vi "Button Pressed.vi"(8 "error in (no error)":errorcluster, 9 "Data":variant, 10 "Button":T1, 11 "Guardian in":refnum<class "Guardian.lvclass">) -> (0 "error out":errorcluster, 3 "Guardian out":refnum<class "Guardian.lvclass">)   [LabVIEW 2020, in "TALOS.lvlib" / "Guardian.lvlib" / "Guardian.lvclass"]
doc: "This VI execute when a message Button Pressed is invoked from the Guardian Interface (not the GUI, the Interface...)."
uses:
  Guardian.lvclass
  C:/LabVIEW Code/TALOS/builds/Actor Framework PPL/Actor Framework.lvlibp/1abvi3w/vi.lib/ActorFramework/Actor/Actor.lvclass
  C:/LabVIEW Code/TALOS/talos/Ancestor/Ancestor/Ancestor.lvclass
  Buttons_UI.ctl
  Internal uServices/System uServices/Guardian Subpanel/Launch uService Message.ctl
  Guardian Messages/Launch uService Msg/Launch uService Msg.lvclass/Launch uService Msg.ctl
  Ancestor/Ancestor/Ancestor.lvclass/Ancestor.ctl
  Classes/uService List/uService List.lvclass/uService List.ctl
  builds/Actor Framework PPL/Actor Framework.lvlibp/1abvi3w/vi.lib/ActorFramework/Message Enqueuer/Message Enqueuer.lvclass
  Guardian.lvclass/Guardian.ctl
  Guardian Messages/Message to Other Guardian Msg/Message to Other Guardian Msg.lvclass/Message to Other Guardian Msg.ctl
  Guardian Messages/TCP-SV Message Interpreter Msg/TCP-SV Message Interpreter Msg.lvclass/TCP-SV Message Interpreter Msg.ctl
  Git Update Cluster.ctl
  Guardian Messages/Message to uService Msg/Message to uService Msg.lvclass/Message to uService Msg.ctl
  Classes/uService List/Get Queue.vi
  Ancestor/Ancestor/Read ID.vi
  Support VIs/Search Array of Strings.vi
  Guardian Messages/TCP-SV Message Interpreter Msg/Send TCP-SV Message Interpreter.vi
  FGV/Error Memory/Get Error Description.vi
  Support VIs/Get PC name.vi
  Support VIs/Get Class Name.vi
  <vilib>/Utility/error.llb/Clear Errors.vi
  FGV/Error Memory/Error Memory Core.vi
  <vilib>/AdvancedString/Delimited String to 1D String Array.vi
  FGV/Error Memory/Error Crt Lvl checker.vi
  FGV/Error Memory/Error Memory Core.vi/40c8088d-b597-4017-91af-faa98e00292e.vi
  FGV/Error Memory/Error Memory Core.vi/d4a3ab98-063c-4e44-b43d-fbdcfe6c2be2.vi
  builds/Actor Framework PPL/Actor Framework.lvlibp/1abvi3w/vi.lib/ActorFramework/Message Enqueuer/Enqueue.vi
  Support VIs/Global Memory.vi
  <vilib>/Utility/LVClass/Get LV Class Name.vi
  Support VIs/Is in Packed Library.vi
  Support VIs/TALOS Root path.vi
  Support VIs/Read CSV worksheet.vi
  Support VIs/Global Constants.vi
  <vilib>/Utility/error.llb/General Error Handler.vi
  Support VIs/Error Log.vi
  Support VIs/Circus Critical PCs List.vi
  Extract uService List from CSV.vi
  Guardian Messages/Launch uService Msg/Launch uService Msg.lvclass
  Ancestor/Ancestor/Ancestor.lvclass
  <vilib>/Comparison/Equal/Equal Functor/Equal Functor.lvclass
  Guardian Messages/Message to Other Guardian Msg/Message to Other Guardian Msg.lvclass
  Guardian Messages/TCP-SV Message Interpreter Msg/TCP-SV Message Interpreter Msg.lvclass
  Guardian Messages/Message to uService Msg/Message to uService Msg.lvclass
  Guardian Messages/I Exist Msg/I Exist Msg.lvclass
  Classes/Guardian List/Guardian List.lvclass
  Classes/uService List/uService List.lvclass
  builds/Actor Framework PPL/Actor Framework.lvlibp/1abvi3w/vi.lib/ActorFramework/Actor/Actor.lvclass
  builds/Actor Framework PPL/Actor Framework.lvlibp/1abvi3w/vi.lib/ActorFramework/Stop Msg/Stop Msg.lvclass
  TALOS.lvlib
  Internal uServices/System uServices/Guardian Subpanel/Guardian Subpanel.lvclass
  C:/LabVIEW Code/TALOS/talos/Guardian/Guardian/Guardian.lvclass
  Guardian Messages/Button Pressed Msg/Button Pressed Msg.lvclass
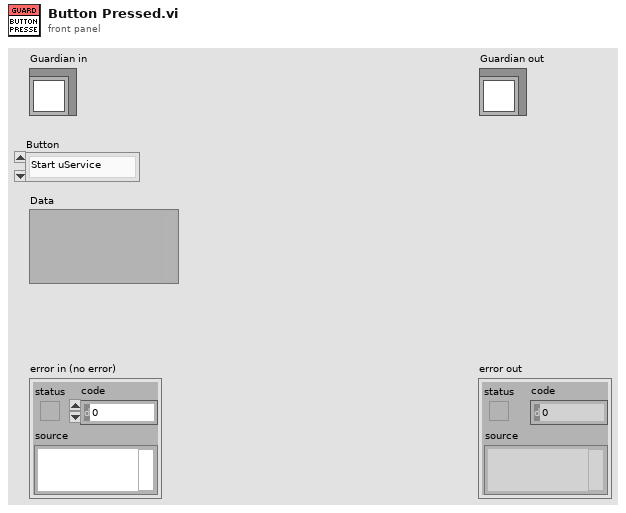
[diagram p1: front panel]
types:
  T1 = typedef "TALOS.lvlib/Guardian.lvlib/Guardian.lvclass/Buttons_UI.ctl" = enum16{"Start uService", "Kill uService", "Stop uService", "Stop", "Start online checks", "Stop online checks", "Send Pat to all GDs", "Reload INI files", "Update from GIT", "RUN", "Reset ABORT", "Check Bearer", "Send I Exist", "Change Run Config", "Add uSs from Config", "Realign uSs from Config", "Send Run Config to GD"}
  T2 = typedef "TALOS.lvlib/Guardian Subpanel.lvlib/Guardian Subpanel.lvclass/Launch uService Message.ctl" = cluster{"uService Class Name":string, "uService ID":string}
  T3 = typedef "TALOS.lvlib/Guardian.lvlib/Guardian.lvclass/Git Update Cluster.ctl" = cluster{"branch name":string, "include critical PCs":bool, "update from git":bool}
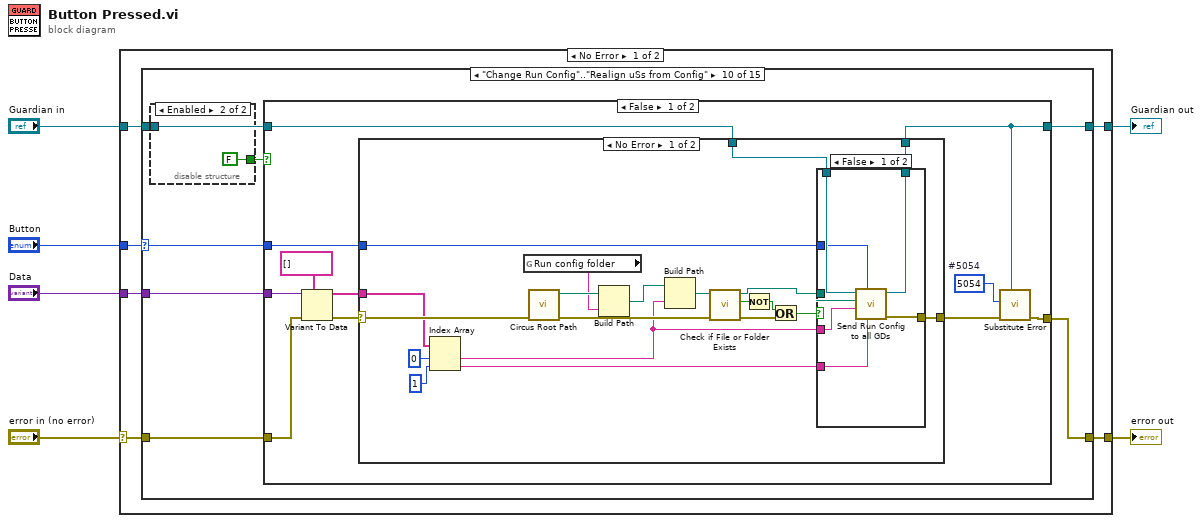
[diagram p0: block diagram]
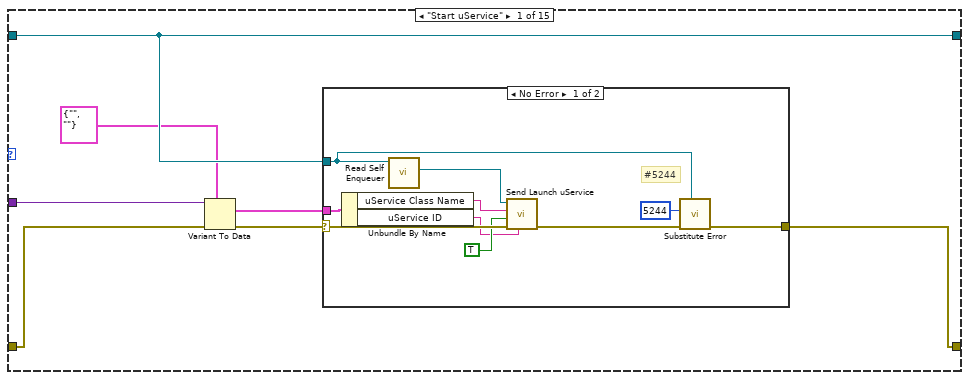
[diagram p2: hidden frame]
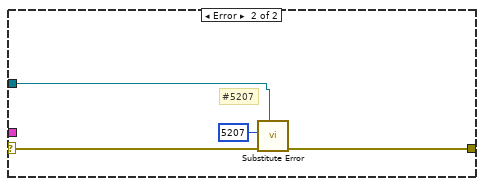
[diagram p3: hidden frame]
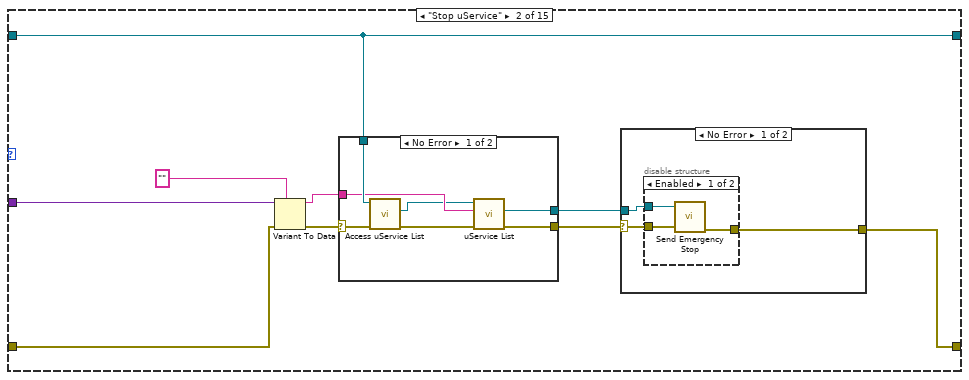
[diagram p4: hidden frame]
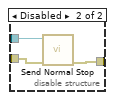
[diagram p5: hidden frame]
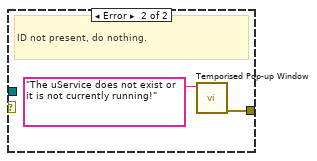
[diagram p6: hidden frame]
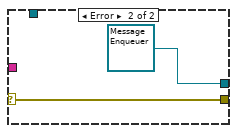
[diagram p7: hidden frame]
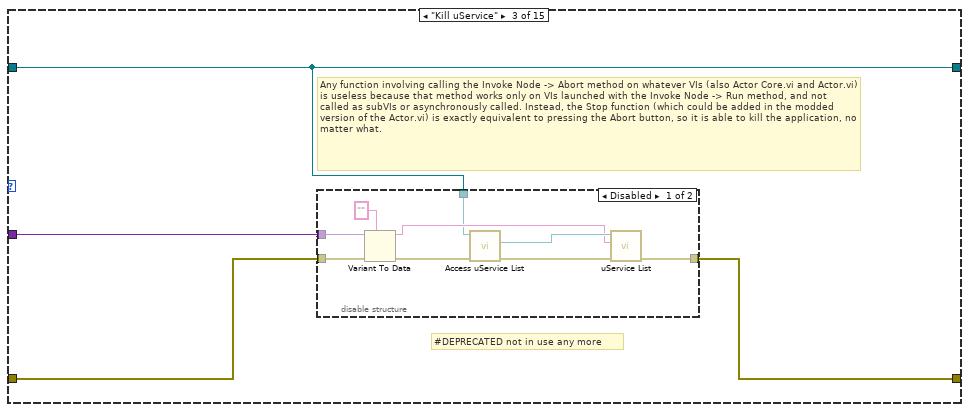
[diagram p8: hidden frame]
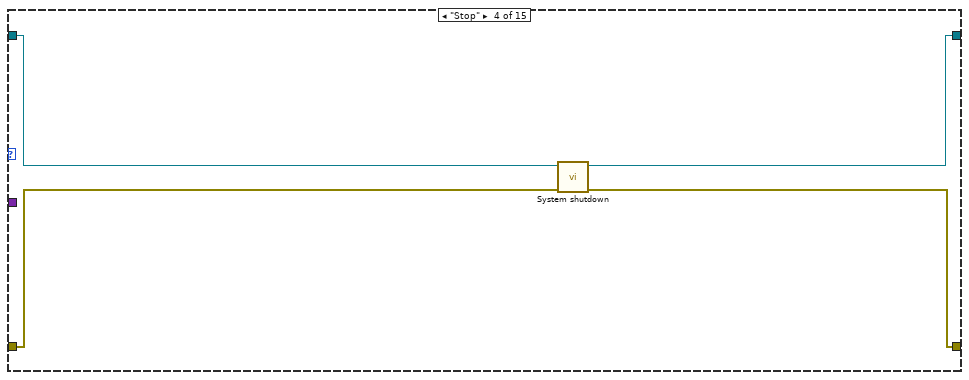
[diagram p10: hidden frame]
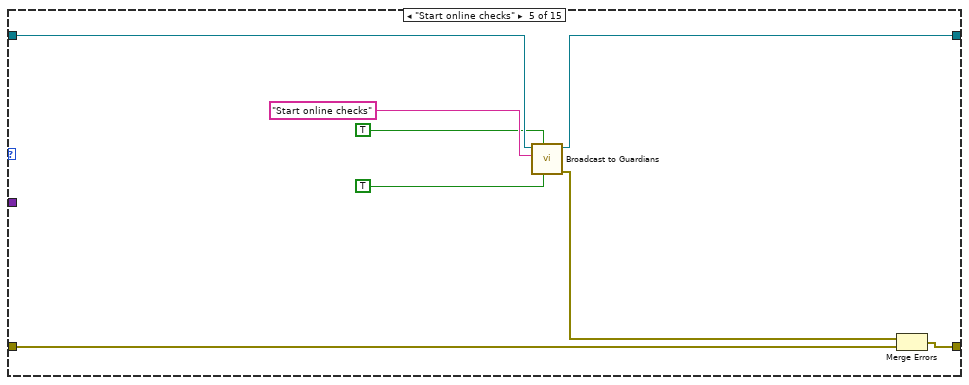
[diagram p11: hidden frame]
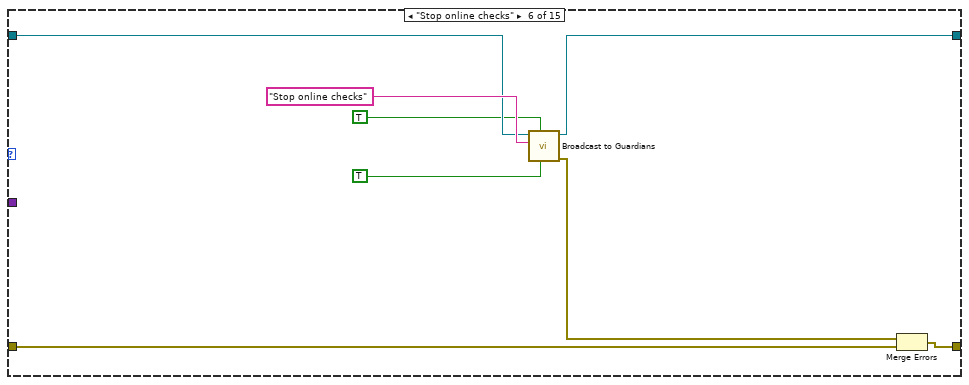
[diagram p12: hidden frame]
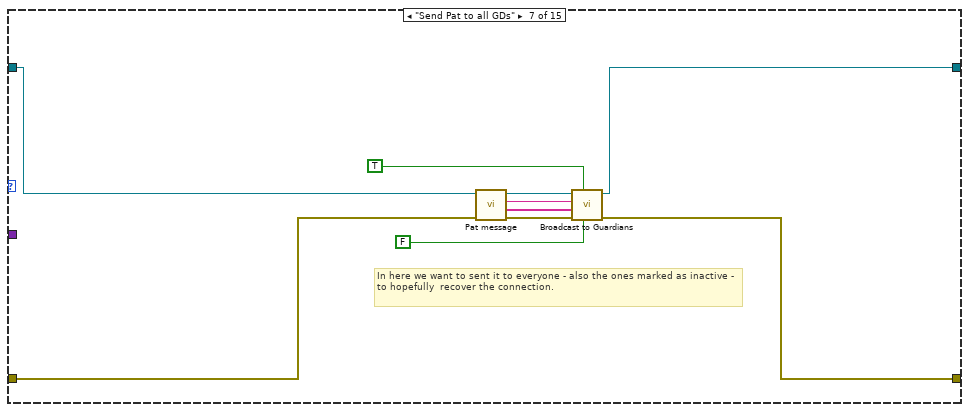
[diagram p13: hidden frame]
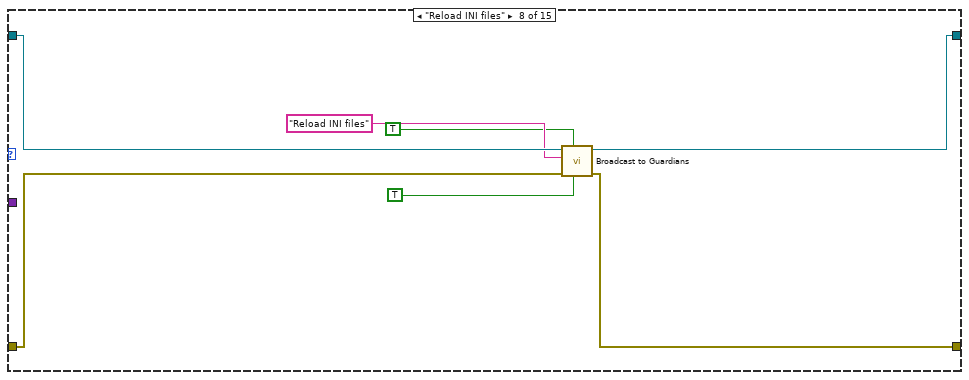
[diagram p14: hidden frame]
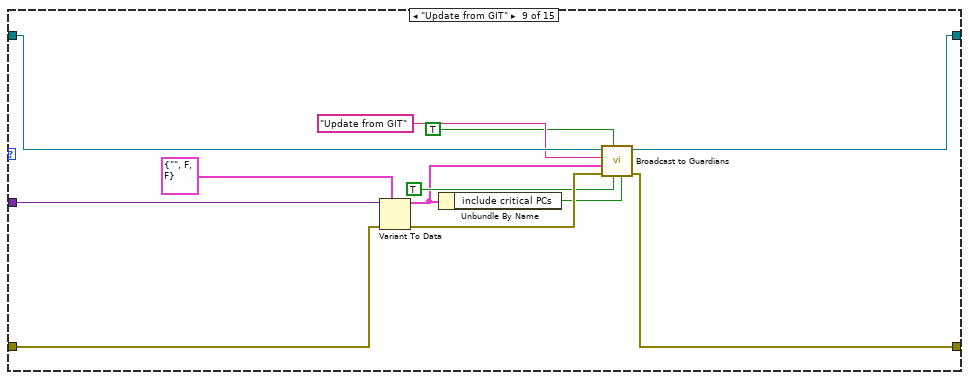
[diagram p15: hidden frame]
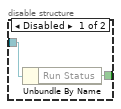
[diagram p16: hidden frame]
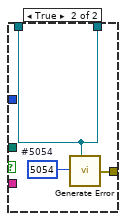
[diagram p17: hidden frame]
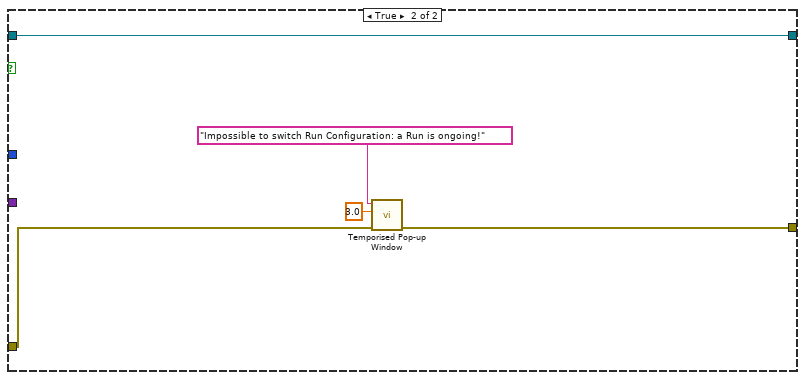
[diagram p19: hidden frame]
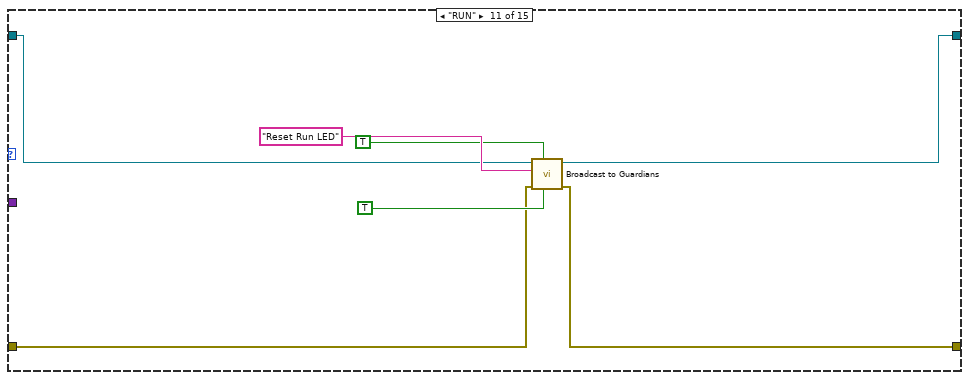
[diagram p20: hidden frame]
diagram:
  n1 = case shown="No Error" "error in (no error)" {
    selector: "error in (no error)" -> [w11 w234]
    tunnel: [w12 w234] -> w5
    tunnel: "Button" -> [w10 _]
    tunnel: [w9 w235] -> w3
    tunnel: "Guardian in" -> [w8 w235]
    tunnel: "Data" -> [w7 _]
    frame No Error {
      n2 = case shown="\"Change Run Config\"..\"Realign uSs from Config\"" w10 {
        selector: w10 -> [_ _ _ _ _ _ _ _ _ w126 _ _ _ _ _]
        tunnel: [w14 w34 w64 w80 w86 w95 w97 w108 w123 w130 w184 w196 w197 w212 w218] -> w12
        tunnel: w11 -> [w18 w41 w65 w77 w87 w96 w99 w110 w122 w132 w185 w195 _ w209 w222]
        tunnel: [w15 w38 w63 w79 w84 w91 w98 w111 w124 w129 w186 w193 w199 w213 w215] -> w9
        tunnel: w8 -> [w15 w38 w63 w78 w88 w92 w100 w112 w125 w128 w187 w194 w199 w213 w219]
        tunnel: w7 -> [w19 w42 w66 _ _ _ _ _ w121 w131 _ _ _ _ w224]
        frame "Start uService" {
          n3 = Variant To Data(error in=w18, type=T2 {"uService Class Name"="", "uService ID"=""}, Variant=w19) -> (data=w17:T2, error out=w16:errorcluster)
          n4 = case shown="No Error" w16 {
            selector: w16 -> [w29 w32]
            tunnel: w17 -> [w22 _]
            tunnel: w15 -> [w24 w31]
            tunnel: [w23 w30] -> w14
            frame No Error {
              # "#5244"
              n5 = Unbundle By Name(w22) -> ("uService Class Name"=w21:string, "uService ID"=w20:string)
              n6 = call "Read Self Enqueuer.vi"("Actor"=w24) -> ("Self Enqueuer"=w28:refnum<class "Message Enqueuer.lvclass">)  [unwired: 10 in]
              n7 = call "Send Launch uService.vi"("uService ID"=w20, "error in (no error)"=w29, "GUI?"=TRUE, "uService Class Name"=w21, "Message Enqueuer"=w28) -> ("error out"=w25:errorcluster)  [unwired: 5 in, 1 out]
              n8 = call "Substitute Error.vi"("LabVIEW Object"=w24, "error in (no error)"=w25, "Error Code"=5244) -> ("error out"=w23:errorcluster)  [unwired: 8 in]
            }
            frame Error {
              # "#5207"
              n9 = call "Substitute Error.vi"("LabVIEW Object"=w31, "error in (no error)"=w32, "Error Code"=5207) -> ("error out"=w30:errorcluster)  [unwired: 8 in]
            }
          }
        }
        frame "Stop uService" {
          n10 = Variant To Data(error in=w41, type="", Variant=w42) -> (data=w37:string, error out=w39:errorcluster)
          n11 = case shown="No Error" w39 {
            selector: w39 -> [w60 w62]
            tunnel: w38 -> [w58 _]
            tunnel: w37 -> [w57 _]
            tunnel: [w55 w62] -> w36
            tunnel: [w54 refnum<class "Message Enqueuer.lvclass"> refnum ("uService Queue")] -> w35
            frame No Error {
              n12 = call-dynamic "Access uService List.vi"("error in (no error)"=w60, "Ancestor in"=w58) -> ("error out"=w59:errorcluster, "uService List out"=w56:refnum<class "uService List.lvclass">)  [unwired: 7 in, 1 out]
              n13 = call-poly "uService List.vi"("error in (no error)"=w59, "ID"=w57, "uService List in"=w56) -> ("error out"=w55:errorcluster, "uService Queue"=w54:refnum<class "Message Enqueuer.lvclass">)  [unwired: 6 in, 1 out]
            }
            frame Error {
            }
          }
          n14 = case shown="No Error" w36 {
            selector: w36 -> [w43 _]
            tunnel: w35 -> [w45 _]
            tunnel: [w44 w53] -> w34
            frame No Error {
              n15 = disable-structure shown="Enabled" {
                disable-tunnel: w43 -> [w48 w51]
                disable-tunnel: w45 -> [w46 w49]
                disable-tunnel: [w47 w50] -> w44
                frame Enabled {
                  n16 = call "Send Emergency Stop.vi"("error in (no error)"=w48, "Message Enqueuer"=w46) -> ("error out"=w47:errorcluster)  [unwired: 9 in]
                }
                frame Disabled {
                  n17 = call "Send Normal Stop.vi"("error in (no error)"=w51, "Message Enqueuer"=w49) -> ("error out"=w50:errorcluster)  [unwired: 9 in]
                }
              }
            }
            frame Error {
              # "ID not present, do nothing."
              n18 = call "Temporised Pop-up Window.vi"("Text"="The uService does not exist or it is not currently running!") -> ("error out"=w53:errorcluster)  [unwired: 10 in]
            }
          }
        }
        frame "Kill uService" {
          # "#DEPRECATED not in use any more"
          # "Any function involving calling the Invoke Node -> Abort method on whatever VIs (also Actor Core.vi and Actor.vi) is useless because that method works only on VIs launched with the Invoke Node -> Run method, and not called as subVIs or asynchronously called. Instead, the Stop function (which could be added in the modded version of the Actor.vi) is exactly equivalent to pressing the Abort button, so it is able to kill the application, no matter what."
          n19 = disable-structure shown="Disabled" {
            disable-tunnel: w66 -> [w74 _]
            disable-tunnel: w65 -> [w73 w76]
            disable-tunnel: [w72 w76] -> w64
            disable-tunnel: w63 -> [w67 _]
            frame Disabled {
              n20 = Variant To Data(error in=w73, type="", Variant=w74) -> (data=w68:string, error out=w71:errorcluster)
              n21 = call-dynamic "Access uService List.vi"("error in (no error)"=w71, "Ancestor in"=w67) -> ("error out"=w70:errorcluster, "uService List out"=w69:refnum<class "uService List.lvclass">)  [unwired: 7 in, 1 out]
              n22 = call-poly "uService List.vi"("error in (no error)"=w70, "ID"=w68, "uService List in"=w69) -> ("error out"=w72:errorcluster)  [unwired: 6 in, 2 out]
            }
            frame Enabled {
            }
          }
        }
        frame "Stop" {
          n23 = call "System shutdown.vi"("error in (no error)"=w77, "Guardian in"=w78) -> ("error out"=w80:errorcluster, "Guardian out"=w79:refnum<class "Guardian.lvclass">)  [unwired: 8 in]
        }
        frame "Start online checks" {
          n24 = call "Broadcast to Guardians.vi"("Only active ones?"=TRUE, "Local also?"=TRUE, "Message"="Start online checks", "Guardian in"=w88) -> ("error out"=w83:errorcluster, "Guardian out"=w84:refnum<class "Guardian.lvclass">)  [unwired: 6 in]
          n25 = Merge Errors(w83, w87) -> (w86:errorcluster)
        }
        frame "Stop online checks" {
          n26 = call "Broadcast to Guardians.vi"("Only active ones?"=TRUE, "Local also?"=TRUE, "Message"="Stop online checks", "Guardian in"=w92) -> ("error out"=w93:errorcluster, "Guardian out"=w91:refnum<class "Guardian.lvclass">)  [unwired: 6 in]
          n27 = Merge Errors(w93, w96) -> (w95:errorcluster)
        }
        frame "Send Pat to all GDs" {
          # "In here we want to sent it to everyone - also the ones marked as inactive - to hopefully  recover the connection."
          n28 = call "Pat message.vi"("error in (no error)"=w99, "Guardian in"=w100) -> ("error out"=w105:errorcluster, "Data"=w104:string[], "Message name"=w102:string, "Guardian out"=w106:refnum<class "Guardian.lvclass">)  [unwired: 6 in]
          n29 = call "Broadcast to Guardians.vi"("Only active ones?"=FALSE, "Local also?"=TRUE, "error in (no error)"=w105, "Data"=w104, "Message"=w102, "Guardian in"=w106) -> ("error out"=w97:errorcluster, "Guardian out"=w98:refnum<class "Guardian.lvclass">)  [unwired: 4 in]
        }
        frame "Reload INI files" {
          n30 = call "Broadcast to Guardians.vi"("Only active ones?"=TRUE, "Local also?"=TRUE, "error in (no error)"=w110, "Message"="Reload INI files", "Guardian in"=w112) -> ("error out"=w108:errorcluster, "Guardian out"=w111:refnum<class "Guardian.lvclass">)  [unwired: 5 in]
        }
        frame "Update from GIT" {
          n31 = Variant To Data(error in=w122, type=T3 {"branch name"="", "include critical PCs"=FALSE, "update from git"=FALSE} ("Git update cluster"), Variant=w121) -> (data=w114:T3, error out=w120:errorcluster)
          n32 = Unbundle By Name(w114) -> ("include critical PCs"=w115:bool)
          n33 = call "Broadcast to Guardians.vi"("Critical PCs also?"=w115, "Only active ones?"=TRUE, "Local also?"=TRUE, "error in (no error)"=w120, "Data"=w114, "Message"="Update from GIT", "Guardian in"=w125) -> ("error out"=w123:errorcluster, "Guardian out"=w124:refnum<class "Guardian.lvclass">)  [unwired: 3 in]
        }
        frame "Change Run Config".."Realign uSs from Config" {
          n34 = disable-structure shown="Enabled" {
            disable-tunnel: w128 -> [w134 _]
            disable-tunnel: [w133 FALSE ("Run Status")] -> w127
            frame Disabled {
              n35 = Unbundle By Name(w134) -> ("Run Status"=w133:bool)
            }
            frame Enabled {
            }
          }
          n36 = case shown="False" w127 {
            tunnel: w128 -> [w146 w179]
            tunnel: w132 -> [w145 w183]
            tunnel: w131 -> [w144 _]
            tunnel: [w139 w182] -> w130
            tunnel: [w138 w179] -> w129
            tunnel: w126 -> [w136 _]
            frame False {
              w137 = 5054  # #5054
              n37 = Variant To Data(error in=w145, type=string[] [], Variant=w144) -> (data=w141:string[], error out=w142:errorcluster)
              n38 = case shown="No Error" w142 {
                selector: w142 -> [w161 w178]
                tunnel: w146 -> [w166 w177]
                tunnel: [w165 w177] -> w138
                tunnel: [w154 w178] -> w140
                tunnel: w141 -> [w153 _]
                tunnel: w136 -> [w152 _]
                frame No Error {
                  n39 = Index Array(array=w153, index #1=0 ("index"), index #2=1 ("index")) -> (element #1=w150:string, element #2=w147:string)
                  n40 = global read "Global Constants.vi" "Run config folder"() -> (w162:string)
                  n41 = call "Circus Root Path.vi"("error in (no error)"=w161) -> ("error out"=w159:errorcluster, "Circus Root Path"=w163:path)  [unwired: 9 in]
                  n42 = Build Path(base path=w163, name or relative path=w162) -> (appended path=w164:path)
                  n43 = Build Path(base path=w164, name or relative path=w150) -> (appended path=w160:path)
                  n44 = call <vilib>:"Check if File or Folder Exists.vi"("error in (no error)"=w159, "path"=w160) -> ("error out"=w158:errorcluster, "file or folder exists?"=w157:bool, "dup path"=w151:path)  [unwired: 7 in]
                  n45 = Not(x=w157) -> (.not. x?=w156:bool)
                  n46 = Or(x=w156, y=w158) -> (x .or. y?=w155:bool)
                  n47 = case shown="False" w155 {
                    tunnel: w166 -> [w173 w176]
                    tunnel: [w172 w176] -> w165
                    tunnel: [w171 w175] -> w154
                    tunnel: w150 -> [w168 _]
                    tunnel: w152 -> [w170 _]
                    tunnel: w151 -> [w169 _]
                    tunnel: w147 -> [w167 _]
                    frame False {
                      n48 = call "Send Run Config to all GDs.vi"("Guardian ID or ALL"=w167, "Button"=w170, "Run Config Name"=w168, "CSV Path"=w169, "Guardian in"=w173) -> ("error out"=w171:errorcluster, "Guardian out"=w172:refnum<class "Guardian.lvclass">)  [unwired: 5 in]
                    }
                    frame True {
                      w174 = 5054  # #5054
                      n49 = call "Generate Error.vi"("Class"=w176, "Error Code"=w174) -> ("error out"=w175:errorcluster)  [unwired: 5 in]
                    }
                  }
                }
                frame Error {
                }
              }
              n50 = call "Substitute Error.vi"("LabVIEW Object"=w138, "error in (no error)"=w140, "Error Code"=w137) -> ("error out"=w139:errorcluster)  [unwired: 8 in]
            }
            frame True {
              n51 = call "Temporised Pop-up Window.vi"("error in (no error)"=w183, "Timeout"=3.0, "Text"="Impossible to switch Run Configuration: a Run is ongoing!") -> ("error out"=w182:errorcluster)  [unwired: 8 in]
            }
          }
        }
        frame "RUN" {
          n52 = call "Broadcast to Guardians.vi"("Only active ones?"=TRUE, "Local also?"=TRUE, "error in (no error)"=w185, "Message"="Reset Run LED", "Guardian in"=w187) -> ("error out"=w184:errorcluster, "Guardian out"=w186:refnum<class "Guardian.lvclass">)  [unwired: 5 in]
        }
        frame "Reset ABORT" {
          n53 = call "Raise or Lower Abort.vi"("error in (no error)"=w195, "Sender"="local", "New Abort Value"=FALSE, "Guardian in"=w194) -> ("error out"=w196:errorcluster, "Guardian out"=w193:refnum<class "Guardian.lvclass">)  [unwired: 6 in]
        }
        frame "Check Bearer" {
          # "#5244"
          n54 = Unbundle By Name(w199) -> ("GD Subpanel ID"=w206:string, "Bearer"=w204:string)
          n55 = call "Read Self Enqueuer.vi"("Actor"=w199) -> ("Self Enqueuer"=w208:refnum<class "Message Enqueuer.lvclass">)  [unwired: 10 in]
          n56 = call "Date n Time.vi"() -> ("Date & Time"=w202:string)  [unwired: 5 in]
          n57 = call <vilib>:"Space Constant.vi"() -> ("String"=w203:string)
          n58 = Concatenate Strings(w204, w203, w202) -> (w201:string)
          n59 = call "Send Message to uService.vi"("uService ID"=w206, "Message"="Update Bearer", "Data"=w201, "Locale?"=TRUE, "Message Enqueuer"=w208) -> ("error out"=w198:errorcluster)  [unwired: 5 in, 1 out]
          n60 = call "Substitute Error.vi"("LabVIEW Object"=w199, "error in (no error)"=w198, "Error Code"=5244) -> ("error out"=w197:errorcluster)  [unwired: 8 in]
        }
        frame "Send I Exist" {
          # "#5244"
          n61 = call "Read Self Enqueuer.vi"("Actor"=w213) -> ("Self Enqueuer"=w211:refnum<class "Message Enqueuer.lvclass">)  [unwired: 10 in]
          n62 = call "Send I Exist.vi"("error in (no error)"=w209, "Message Enqueuer"=w211) -> ("error out"=w210:errorcluster)  [unwired: 8 in, 1 out]
          n63 = call "Substitute Error.vi"("LabVIEW Object"=w213, "error in (no error)"=w210, "Error Code"=5244) -> ("error out"=w212:errorcluster)  [unwired: 8 in]
        }
        frame "Send Run Config to GD" {
          w217 = 5059  # #5059
          n64 = Variant To Data(error in=w222, type="", Variant=w224) -> (data=w220:string, error out=w223:errorcluster)
          n65 = case shown="No Error" w223 {
            selector: w223 -> [_ w232]
            tunnel: w220 -> [w230 _]
            tunnel: w219 -> [w226 w233]
            tunnel: [w226 w233] -> w215
            tunnel: [w227 w232] -> w216
            frame No Error {
              # "GD ID"
              n66 = Unbundle By Name(w226) -> ("Name"=w231:string)
              n67 = Build Array(w231, w230) -> (w228:string[])
              n68 = call "Read Self Enqueuer.vi"("Actor"=w226) -> ("Self Enqueuer"=w225:refnum<class "Message Enqueuer.lvclass">)  [unwired: 10 in]
              n69 = call "Send Button Pressed.vi"("Data"=w228, "Button"=Buttons_UI."Add uSs from Config", "Message Enqueuer"=w225) -> ("error out"=w227:errorcluster)  [unwired: 7 in, 1 out]
            }
            frame Error {
            }
          }
          n70 = call "Substitute Error.vi"("LabVIEW Object"=w215, "error in (no error)"=w216, "Error Code"=w217) -> ("error out"=w218:errorcluster)  [unwired: 8 in]
        }
      }
    }
    frame Error {
    }
  }
  "error out" <- w5
  "Guardian out" <- w3
